vi "Test MQTT-6.0.0-2.vi"(8 "error in (no error)":errorcluster, 11 "Connection":refnum<class "Connection.lvclass">) -> (0 "error out":errorcluster, 3 "Connection":refnum<class "Connection.lvclass">)   [LabVIEW 2013]
uses:
  <vilib>/LabVIEW Open Source Project/Connection/Connection/Connection.lvclass
  <vilib>/LabVIEW Open Source Project/MQTT Control Packets/Control Packets/ControlPacket/Control Packet Type -- enum.ctl
  <vilib>/LabVIEW Open Source Project/Connection/Connection.Websockets/Connection.WS.lvclass
  <vilib>/addons/_JKI Toolkits/Caraya/classes/Test/Test.lvclass
  <vilib>/LabVIEW Open Source Project/MQTT Control Packets/Control Packets/CONNECT/CONNECT.lvclass
  <vilib>/LabVIEW Open Source Project/MQTT Control Packets/Control Packets/ControlPacket/ControlPacket.lvclass
  <vilib>/LabVIEW Open Source Project/MQTT Control Packets/Control Packets/DISCONNECT/DISCONNECT.lvclass
  <vilib>/addons/_JKI Toolkits/Caraya/classes/Assert/Assert.lvclass
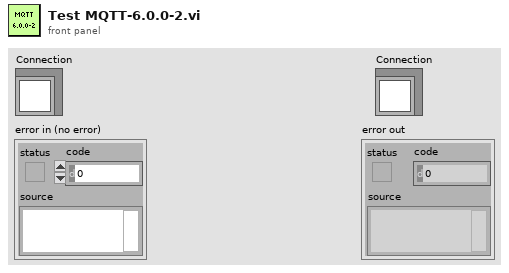
[diagram p1: front panel]
types:
  T1 = typedef "MQTT_Control_Packets.lvlib/ControlPacket.lvclass/Control Packet Type -- enum.ctl" = enum16{"Reserved", "CONNECT", "CONNACK", "PUBLISH", "PUBACK", "PUBREC", "PUBREL", "PUBCOMP", "SUBSCRIBE", "SUBACK", "UNSUBSCRIBE", "UNSUBACK", "PINGREQ", "PINGRESP", "DISCONNECT", "AUTH"}
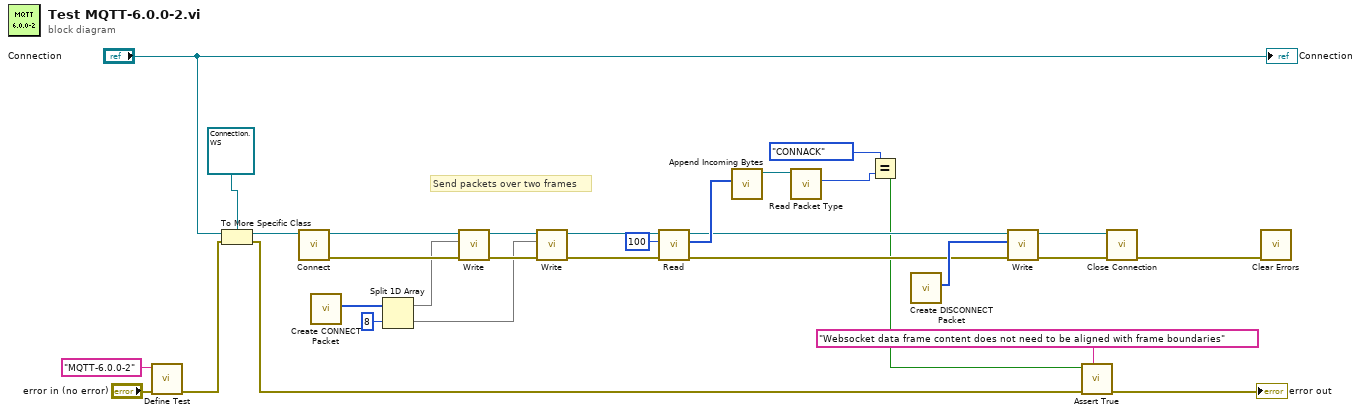
[diagram p0: block diagram]
diagram:
  # "Send packets over two frames"
  n1 = call <vilib>:"Define Test.vi"("error in (no error)"="error in (no error)", "Label (VI Title)"="MQTT-6.0.0-2") -> ("error out"=w24:errorcluster)  [unwired: 9 in]
  n2 = To More Specific Class(target class=refnum<class "Connection.WS.lvclass"> refnum ("Connection.WS in"), reference="Connection", error in=w24) -> (specific class reference=w26:refnum<class "Connection.WS.lvclass">, error out=w23:errorcluster)
  n3 = call <vilib>:"Connect.vi"("Connection in"=w26) -> ("error out"=w21:errorcluster, "Connection out"=w22:refnum<class "Connection.WS.lvclass">)  [unwired: 9 in]
  n4 = call <vilib>:"Create CONNECT Packet.vi"() -> ("Bytes Stream"=w12:u8[])  [unwired: 9 in, 2 out]
  n5 = Split 1D Array(array=w12, index=8) -> (first subarray=w13:u8[], second subarray=w14:u8[])
  n6 = call <vilib>:"Write.vi"("error in (no error)"=w21, "Bytes"=w13, "Connection in"=w22) -> ("error out"=w17:errorcluster, "Connection"=w19:refnum<class "Connection.WS.lvclass">)  [unwired: 7 in]
  n7 = call <vilib>:"Write.vi"("error in (no error)"=w17, "Bytes"=w14, "Connection in"=w19) -> ("error out"=w16:errorcluster, "Connection"=w18:refnum<class "Connection.WS.lvclass">)  [unwired: 7 in]
  n8 = call <vilib>:"Read.vi"("error in (no error)"=w16, "bytes to read (100)"=100, "TCPConnection in"=w18) -> ("error out"=w4:errorcluster, "Bytes"=w11:u8[], "TCPConnection out"=w6:refnum<class "Connection.WS.lvclass">)  [unwired: 4 in, 2 out]
  n9 = call <vilib>:"Append Incoming Bytes.vi"("Incoming Packets"=w11) -> ("ControlPacket"=w10:refnum<class "ControlPacket.lvclass">)  [unwired: 7 in, 3 out]
  n10 = call <vilib>:"Read Packet Type.vi"("ControlPacket in"=w10) -> ("Control Packet Type"=w9:T1)  [unwired: 9 in, 1 out]
  n11 = Equal?(x=Control_Packet_Type_--_enum."CONNACK", y=w9) -> (x = y?=w2:bool)
  n12 = call <vilib>:"Create DISCONNECT Packet.vi"() -> ("Bytes Stream"=w7:u8[])  [unwired: 9 in, 2 out]
  n13 = call <vilib>:"Write.vi"("error in (no error)"=w4, "Bytes"=w7, "Connection in"=w6) -> ("error out"=w3:errorcluster, "Connection"=w5:refnum<class "Connection.WS.lvclass">)  [unwired: 7 in]
  n14 = call <vilib>:"Assert True.vi"("Label"="Websocket data frame content does not need to be aligned with frame boundaries", "error in (no error)"=w23, "True?"=w2) -> ("error out"=→"error out":errorcluster)  [unwired: 8 in]
  n15 = call <vilib>:"Close Connection.vi"("error in (no error)"=w3, "Connection in"=w5) -> ("error out"=w27:errorcluster)  [unwired: 8 in, 1 out]
  n16 = call <vilib>:"Clear Errors.vi"("error in (no error)"=w27) -> ()  [unwired: 6 in, 1 out]
  "Connection" <- "Connection"
